vi "Step_Tick.vi"(8 "error in (no error)":errorcluster={"status"=FALSE, "code"=0, "source"="\"\""}, 10 "current time":i64=1500, 11 "StepContext":string) -> (0 "error out":errorcluster={"status"=FALSE, "code"=0, "source"="\"\""}, 2 "status ok":bool, 3 "Updated StepContext and outgoing requests":string)   [LabVIEW 2026]
doc: "INTENT: Cooperative step tick evaluating step duration, condition progress, and timeout limits."
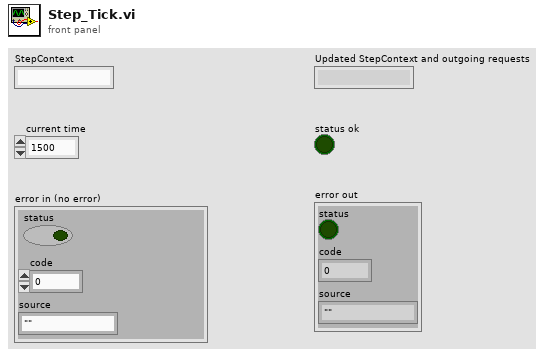
[diagram p1: front panel]
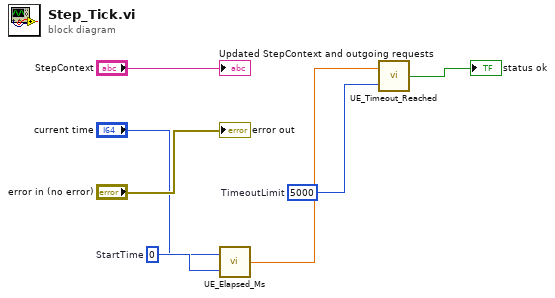
[diagram p0: block diagram]
diagram:
  w5 = i64 5000  # TimeoutLimit
  w4 = i64 0  # StartTime
  n1 = call "UE_Elapsed_Ms.vi"("start_ms"=w4, "now_ms"="current time") -> ("elapsed_ms"=w6:dbl)
  n2 = call "UE_Timeout_Reached.vi"("threshold_ms"=w5, "elapsed_ms"=w6) -> ("reached"=→"status ok":bool)
  "Updated StepContext and outgoing requests" <- "StepContext"
  "error out" <- "error in (no error)"
